vi "SerialDelayRecv.vi"(7 "Timeout":u32=50, 8 "error in (no error)":errorcluster caption="错误输入（无错误）", 11 "Port":refnum<visa-resource-name>) -> (0 "error out":errorcluster caption="错误输出", 2 "Buff":string, 3 "Port out":refnum<visa-resource-name>)   [LabVIEW 2025]
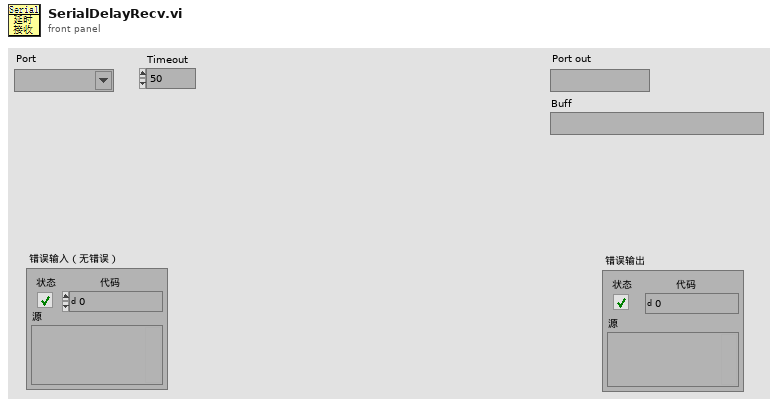
[diagram p1: front panel]
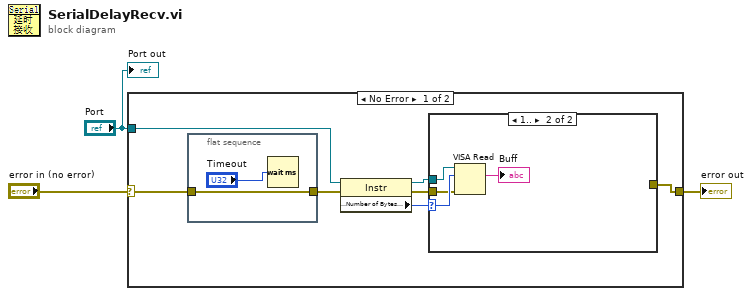
[diagram p0: block diagram]
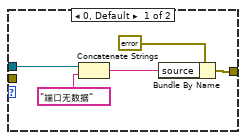
[diagram p2: hidden frame]
diagram:
  n1 = case shown="No Error" "error in (no error)" {
    selector: "error in (no error)" -> [w8 w22]
    tunnel: [w9 w22] -> w3
    tunnel: "Port" -> [w10 _]
    frame No Error {
      n2 = flat-sequence {
        tunnel: [w12] -> w4
        tunnel: w8 -> [w12]
        frame #0 {
          n3 = Wait (ms)(milliseconds to wait="Timeout") -> ()  [unwired: 1 out]
        }
      }
      n4 = property class="Instr"(reference=w10, error in=w4) -> (reference out=w7:refnum<visa-resource-name>, error out=w5:errorcluster, "Serial Settings:Number of Bytes at Serial Port"=w6:u32)
      n5 = case shown="1.." w6 {
        selector: w6 -> [_ w20]
        tunnel: w7 -> [w14 w21]
        tunnel: [w16 _] -> w9
        tunnel: w5 -> [_ w19]
        frame 0, Default {
          n6 = Concatenate Strings(w14, "端口无数据" ("error")) -> (w15:string)
          n7 = Bundle By Name(cluster=errorcluster {"status"=TRUE, "code"=0, "source"=""} ("error"), "source"=w15) -> (w16:errorcluster)
        }
        frame 1.. {
          n8 = VISA Read(VISA resource name=w21, byte count=w20, error in (no error)=w19) -> (read buffer=→"Buff":string)  [unwired: 3 out]
        }
      }
    }
    frame Error {
    }
  }
  "error out" <- w3
  "Port out" <- "Port"
